vi "Eval_SglVar_BulkMode.vi"(8 "error in (no error)":errorcluster, 9 "varValue":dbl[](array[numeric]) format="%#_13g", 11 "muExpr in":refnum<class "mupExpr.lvclass">) -> (0 "error out":errorcluster, 2 "Result":dbl[](array[numeric]), 3 "muExpr out":refnum<class "mupExpr.lvclass">)   [LabVIEW 2015, in "mupExpr.lvclass"]
doc: "Updates the values of the selected single variable then evaluates the expression in bulk mode. Returns the array of results.\n\nIf the expression contains no variables, the input values are ignored.\n\nIf the expression contains more than one variable only the \"Single Variable\" is updated.\n\nIf multiple expressions have been input, the result of the last one in the list is returned."
uses:
  mupExpr.lvclass
  mupExpr.lvclass/mupExpr.ctl
  mupLib/mupCheckError.vi
  <vilib>/Utility/error.llb/Error Cluster From Error Code.vi
  mupLib/mupLib.lvlib
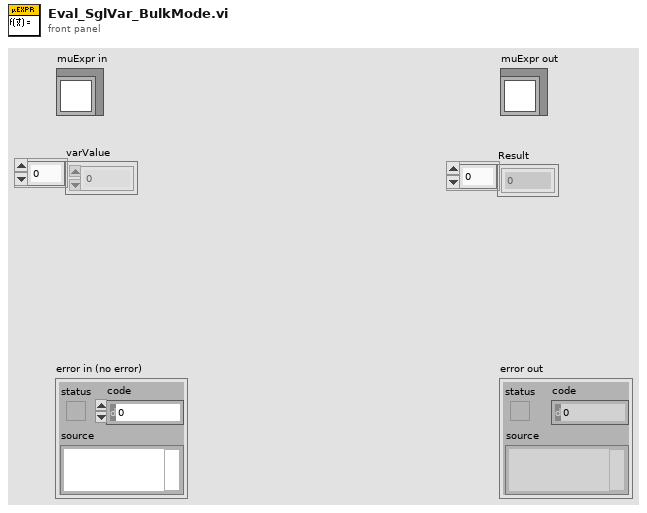
[diagram p1: front panel]
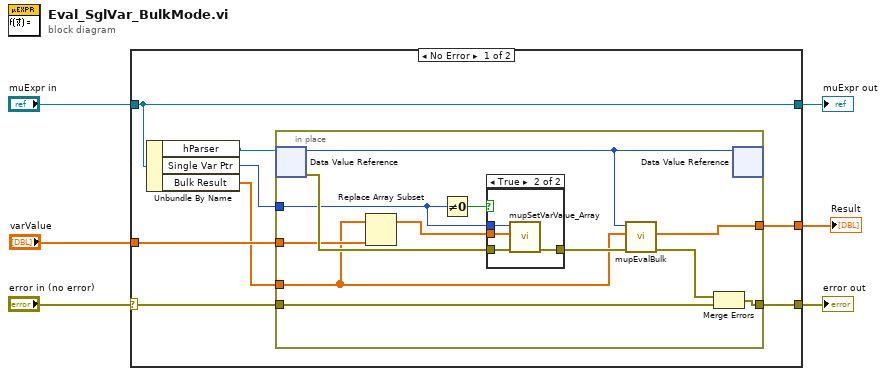
[diagram p0: block diagram]
diagram:
  n1 = case shown="No Error" "error in (no error)" {
    selector: "error in (no error)" -> [w14 w33]
    tunnel: [w12 w33] -> w5
    tunnel: [w7 w32] -> w3
    tunnel: "muExpr in" -> [w7 w32]
    tunnel: "varValue" -> [w13 _]
    tunnel: [w11 _] -> w1
    frame No Error {
      n2 = Unbundle By Name(w7) -> ("hParser"=w10:refnum<data-value>, "Single Var Ptr"=w9:u64, "Bulk Result"=w8:dbl[])
      n3 = in-place {
        in-place-border: w14 -> [w24]
        in-place-border: w13 -> [w21]
        in-place-border: [w22] -> w12
        in-place-border: [w26] -> w11
        in-place-border: w9 -> [w17]
        in-place-border: w8 -> [w16]
        n4 = in-place-dvr #1(w10) -> (w15:u64, w25:errorcluster)
        n5 = Replace Array Subset(array=w16, new element=w21) -> (w19:dbl[])  [unwired: 1 in]
        n6 = Not Equal To 0?(x=w17) -> (x != 0?=w18:bool)
        n7 = case shown="True" w18 {
          tunnel: w25 -> [w27 w31]
          tunnel: [w27 w30] -> w20
          tunnel: w19 -> [_ w29]
          tunnel: w17 -> [_ w28]
          frame False {
          }
          frame True {
            n8 = call "mupSetVarValue_Array.vi"("error in (no error)"=w31, "varValue"=w29, "varPtr in"=w28) -> ("error out"=w30:errorcluster)  [unwired: 7 in, 1 out]
          }
        }
        n9 = call "mupEvalBulk.vi"("error in (no error)"=w20, "a_res"=w16, "hParser in"=w15) -> ("error out"=w23:errorcluster, "results"=w26:dbl[])  [unwired: 6 in, 1 out]
        n10 = Merge Errors(w23, w24) -> (w22:errorcluster)
        n11 = in-place-dvr #1(w15) -> ()  [unwired: 2 out]
      }
    }
    frame Error {
    }
  }
  "error out" <- w5
  "muExpr out" <- w3
  "Result" <- w1
